vi "CIF_Iceoryx_Tag Update Test Cases.vi"() -> (0 "error out":errorcluster, 2 "status":string, 3 "pass":bool)   [LabVIEW 2021]
uses:
  ChannelCommon/typedef/Direction.ctl
  Double/CIF_Iceoryx_Chn_Double.lvclass
  D:/dev/Packages/CIF_Channels_Core/src/Iceorxy_Channels/CIF_Iceoryx_BB/CIF_Iceoryx_BB.lvclass
  D:/dev/Packages/CIF_Channels_Core/src/CIFChannels/CIFChannels.lvclass
  ChannelCommon/typedef/New FIFO Instance Response.ctl
  CIFChannels/CIFChannels.lvclass/CIFChannels.ctl
  U64/CIF_Iceoryx_Chn_U64.lvclass
  I64/CIF_Iceoryx_Chn_I64.lvclass
  CIF_Iceoryx_BB/CIF_Iceoryx_BB.lvclass/CIF_Iceoryx_BB.ctl
  8a10abfc-3488-46de-9eab-28ae7432ccba.vi
  <vilib>/CIF Foundation/CIF Iceoryx/SubVIs/Get Path.vi
  <vilib>/CIF Foundation/CIF Iceoryx/SubVIs/Convert Error.vi
  <vilib>/CIF Foundation/CIF Iceoryx/Refnum/BB Reader from Refnum.vi
  <vilib>/CIF Foundation/CIF Iceoryx/SubVIs/Convert Error Core.vi
  ChannelCommon/ChannelCommon.lvlib
  CIFChannels/CIFChannels.lvclass
  <vilib>/CIF Foundation/CIF Iceoryx/Iceoryx.lvlib
  CIF_Iceoryx_BB/CIF_Iceoryx_BB.lvclass
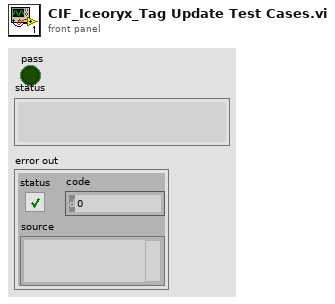
[diagram p1: front panel]
types:
  T1 = typedef "ChannelCommon.lvlib/Direction.ctl" = enum8{"Publisher", "Subscriber"}
  T2 = typedef "ChannelCommon.lvlib/New FIFO Instance Response.ctl" = cluster{"Publisher":string, "Custom Data":u8[]}
  T3 = typedef "Iceoryx.lvlib/BB Refnum.ctl" = cluster{"refnum":u64, "BB":enum8{"bb"}}
  T4 = typedef "Iceoryx.lvlib/BB Reader Refnum.ctl" = cluster{"refnum":u64, "BB Reader":enum8{"bb_reader"}}
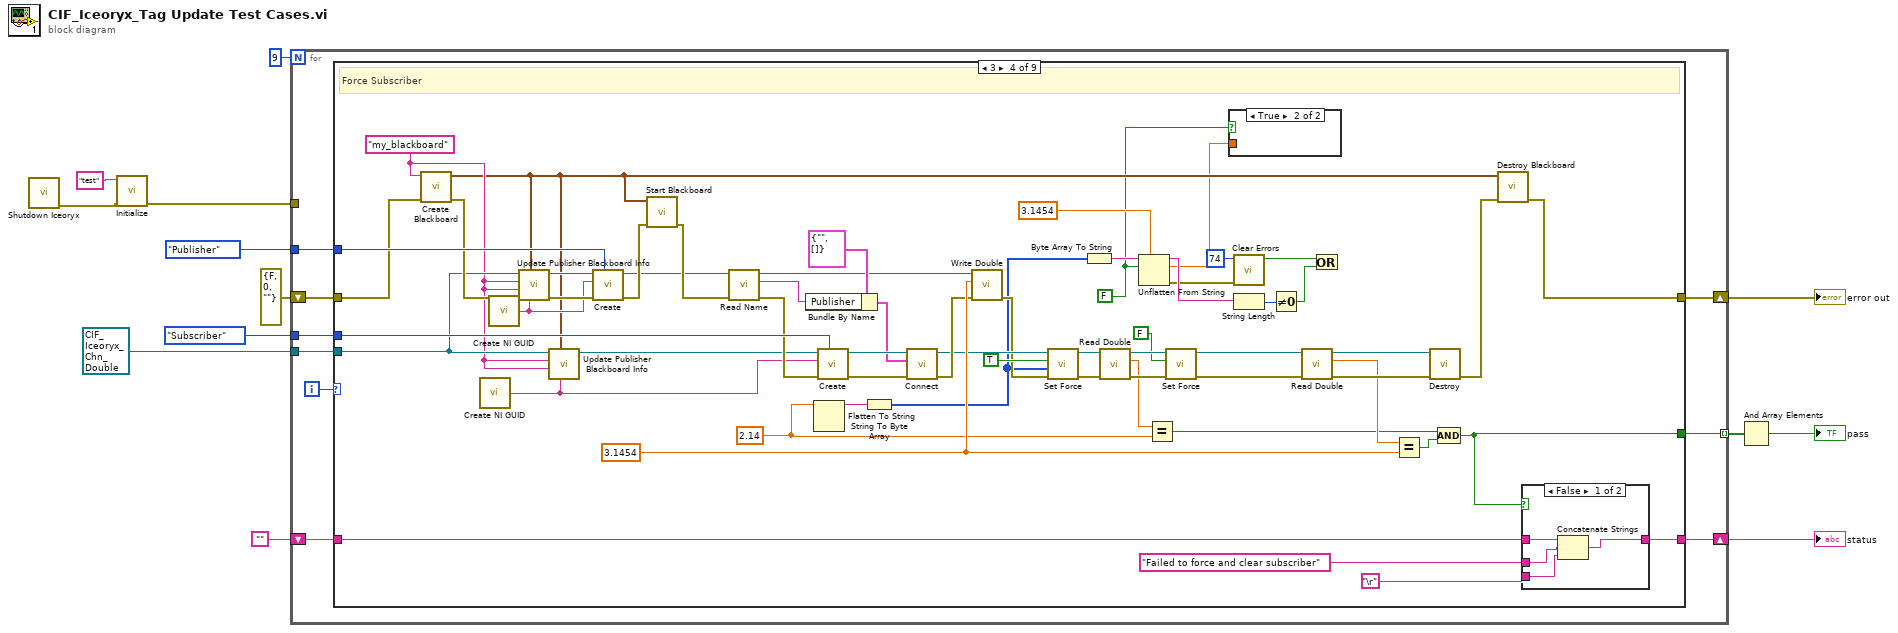
[diagram p0: block diagram]
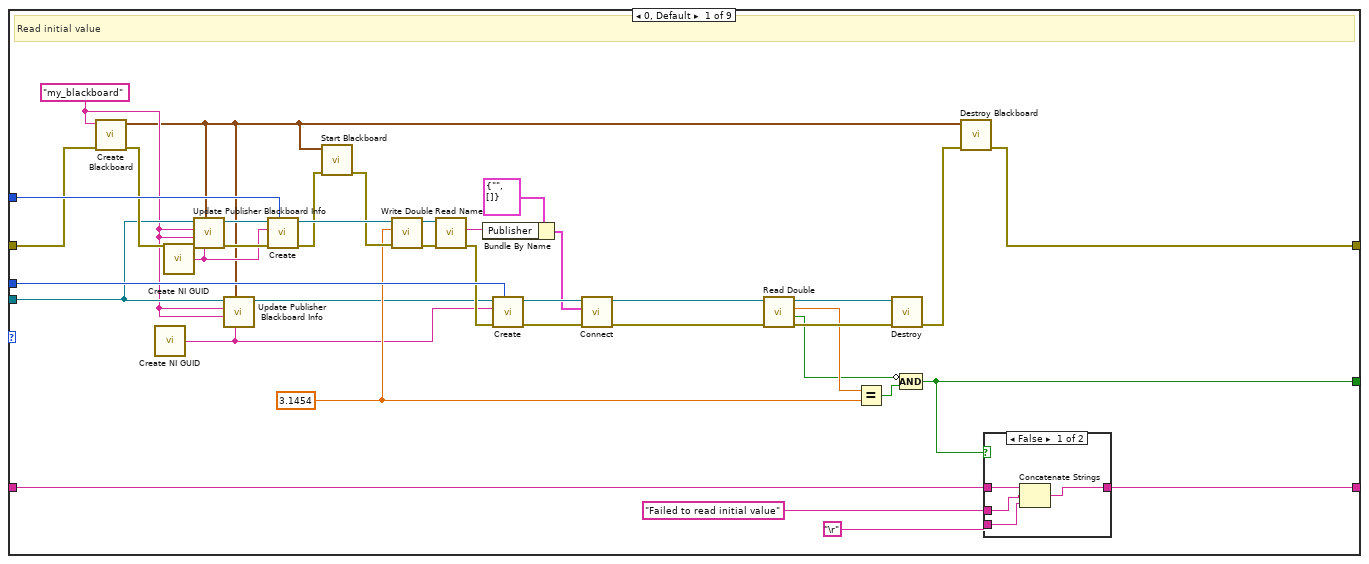
[diagram p2: hidden frame]
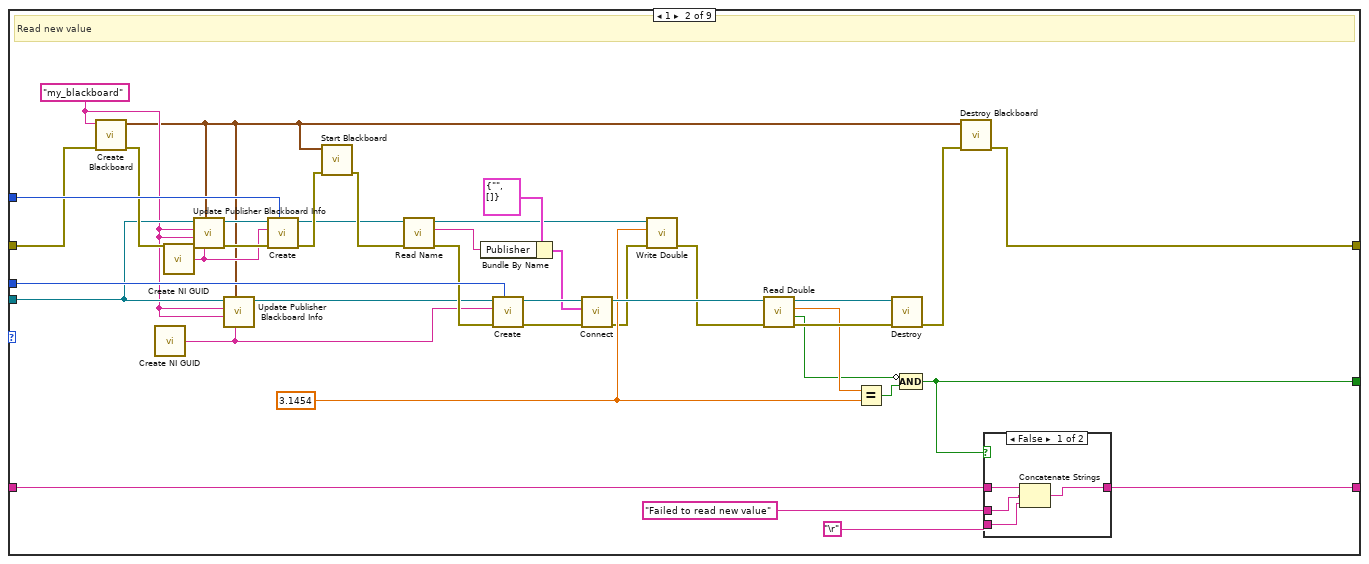
[diagram p4: hidden frame]
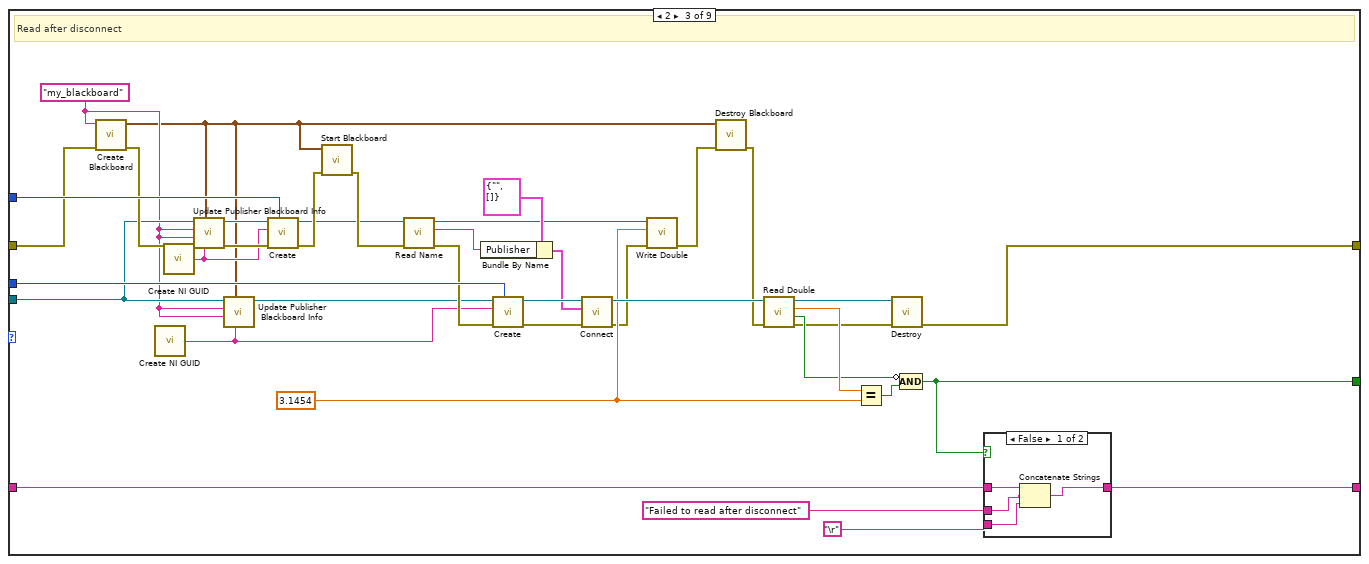
[diagram p6: hidden frame]
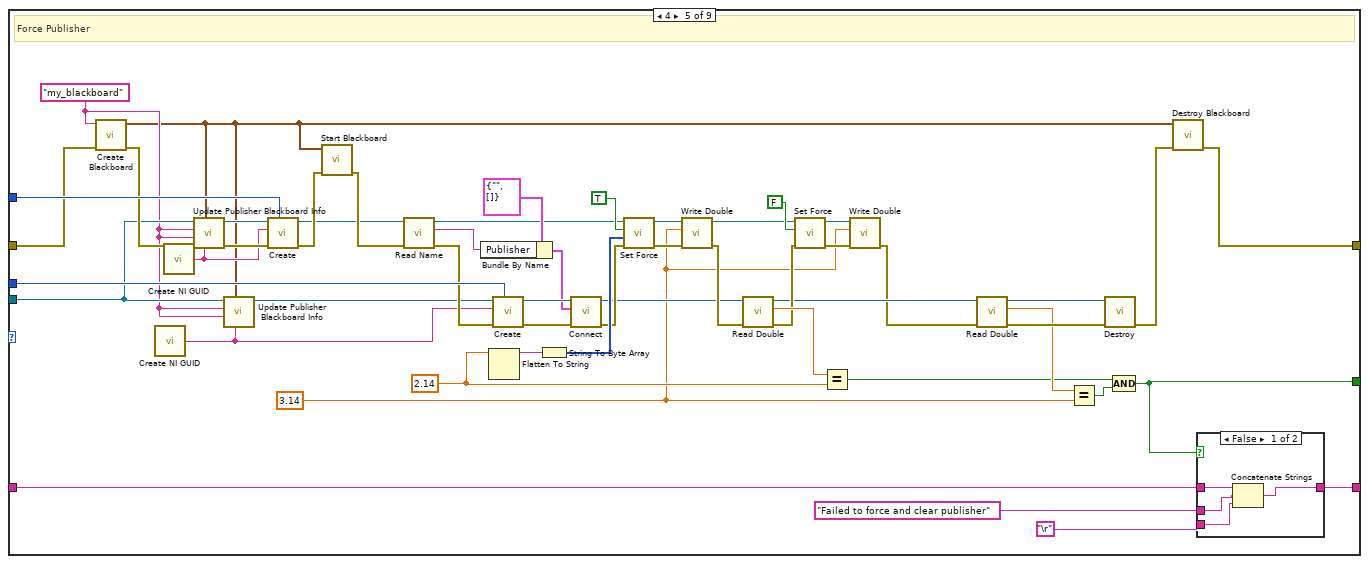
[diagram p10: hidden frame]
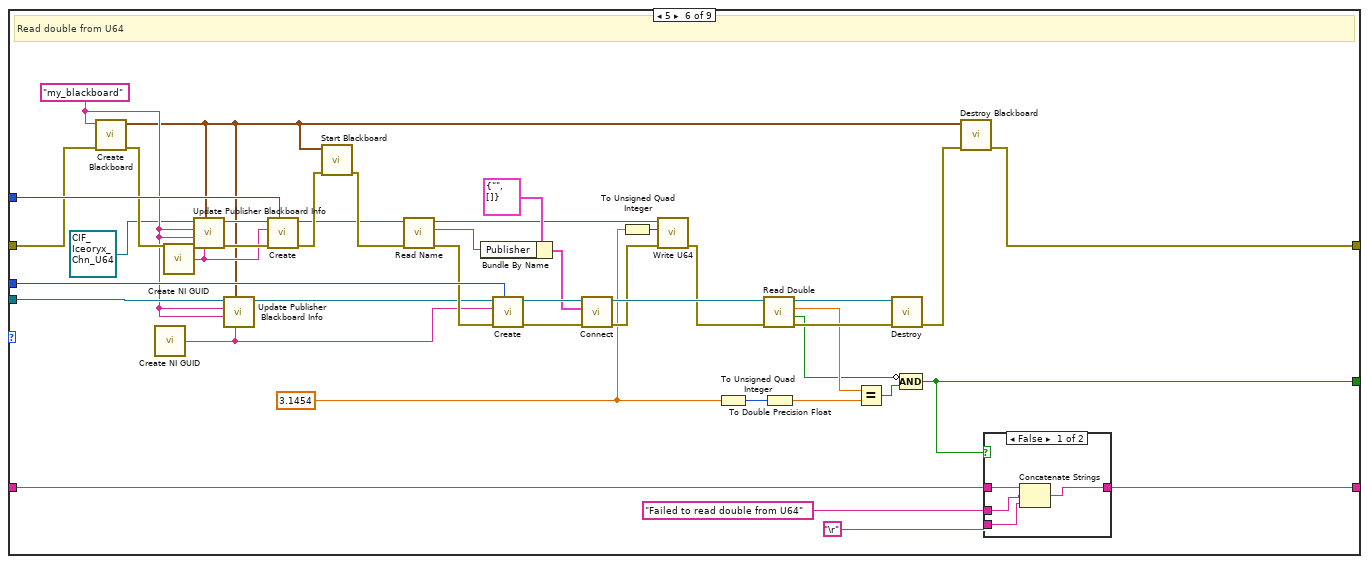
[diagram p12: hidden frame]
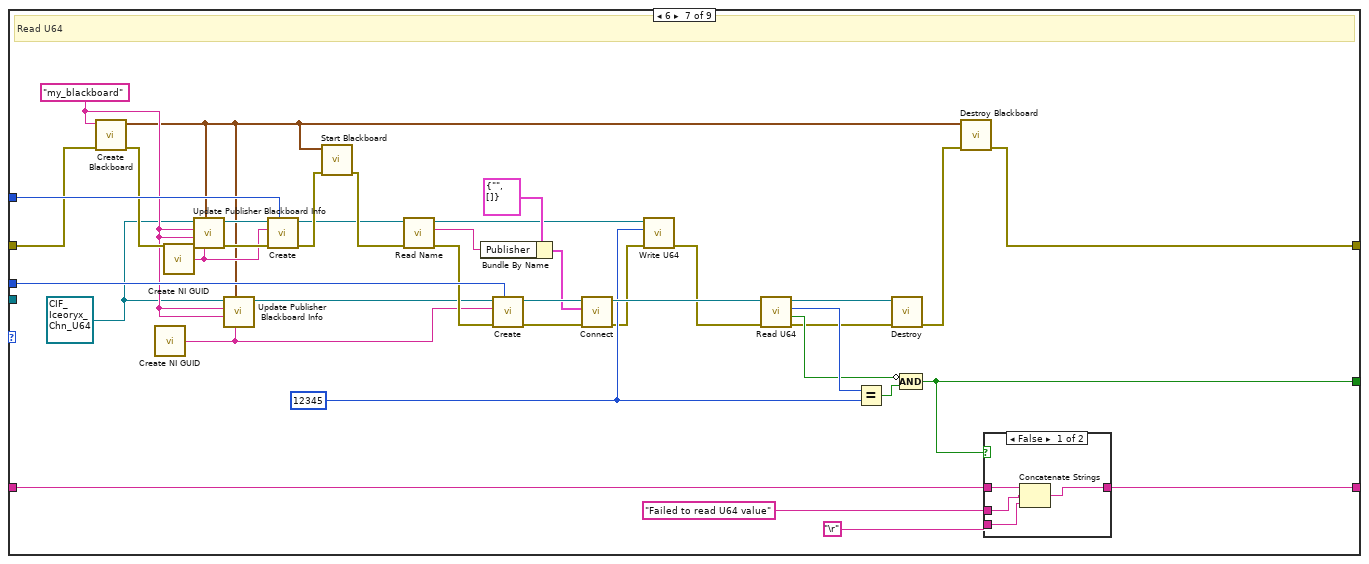
[diagram p14: hidden frame]
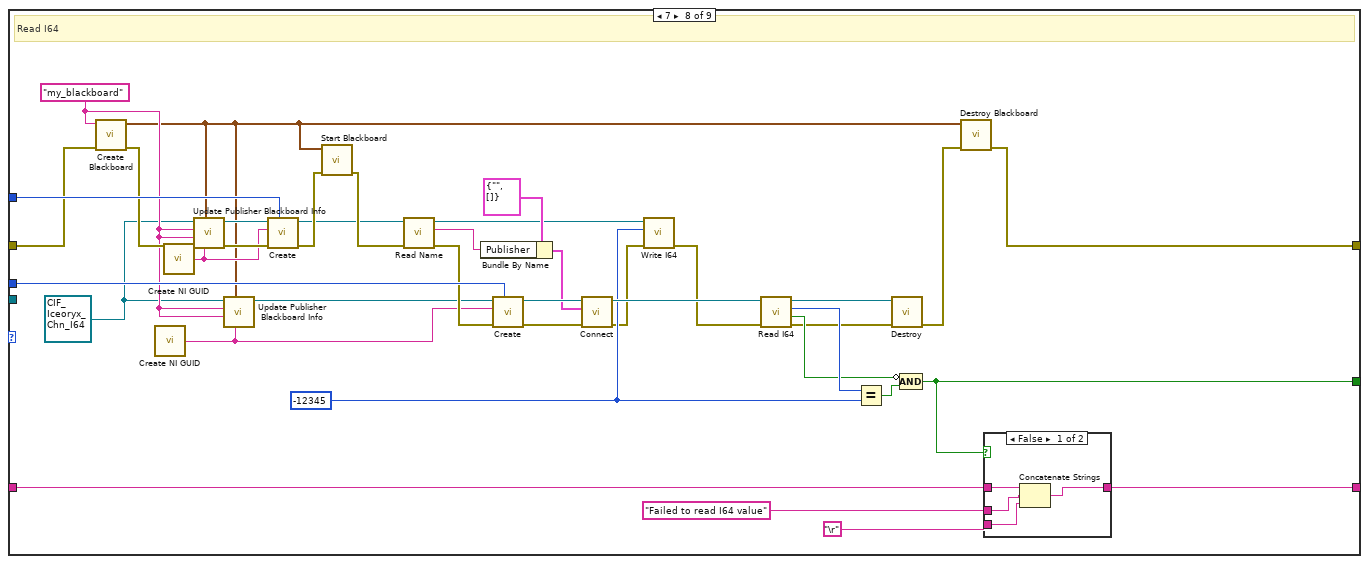
[diagram p16: hidden frame]
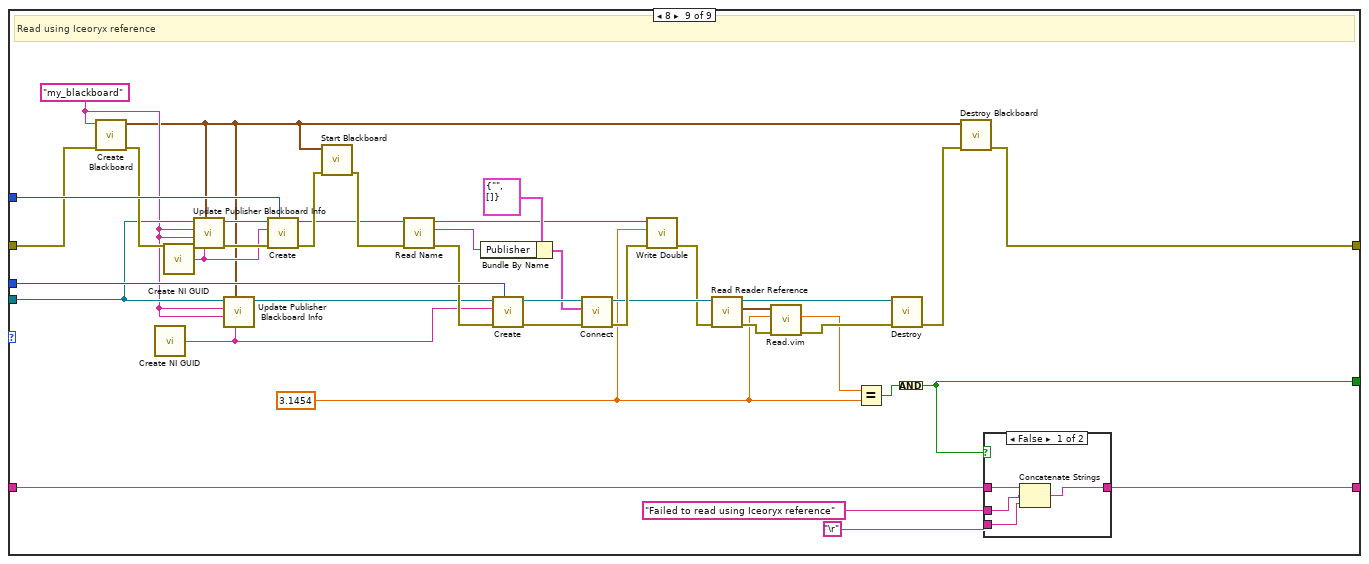
[diagram p18: hidden frame]
diagram:
  n1 = call <vilib>:"Shutdown Iceoryx.vi"() -> ("error out"=w1:errorcluster)  [unwired: 11 in]
  n2 = call <vilib>:"Initialize.vi"("error in (no error)"=w1, "Node name"="test") -> ("error out"=w2:errorcluster)  [unwired: 9 in]
  n3 = for {
    N: 9 -> [_]
    tunnel: [w22] -> w13 mode=indexing
    shift-right: [w20] -> w8
    shift-left: errorcluster {"status"=FALSE, "code"=0, "source"=""} ("error out") -> [w21]
    shift-right: [w17] -> w9
    shift-left: "" -> [w18]
    tunnel: refnum<class "CIF_Iceoryx_Chn_Double.lvclass"> refnum ("CIF_CIPC_Chn_Double.lvclass") -> [w16]
    tunnel: Direction."Publisher" ("Direction") -> [w15]
    tunnel: Direction."Subscriber" ("Direction") -> [w14]
    tunnel: w2 -> [_]
    i -> [w19]
    n4 = case shown="3" w19 {
      tunnel: [w49 w92 w136 w202 w259 w304 w351 w394 w438] -> w22
      tunnel: w21 -> [w42 w86 w130 w197 w254 w298 w346 w389 w433]
      tunnel: [w34 w79 w109 w190 w248 w292 w340 w383 w427] -> w20
      tunnel: w18 -> [w60 w103 w146 w211 w268 w315 w358 w401 w445]
      tunnel: [w59 w102 w145 w210 w267 w314 w357 w400 w444] -> w17
      tunnel: w16 -> [w27 w75 w121 w186 w244 w288 _ _ w423]
      tunnel: w15 -> [w47 w90 w134 w201 w258 w302 w350 w393 w437]
      tunnel: w14 -> [w46 w89 w133 w200 w257 w301 w349 w392 w436]
      frame 0, Default {
        w25 = "my_blackboard" ("Blackboard name")
        w39 = 3.1454
        # "Read initial value"
        n5 = call <vilib>:"Create Blackboard.vi"("error in (no error)"=w42, "Blackboard name"=w25) -> ("error out"=w38:errorcluster, "Blackboard Reference"=w23:T3)  [unwired: 8 in]
        n6 = call <vilib>:"Create NI GUID.vi"() -> ("NI GUID"=w24:string)
        n7 = call <vilib>:"Create NI GUID.vi"() -> ("NI GUID"=w32:string)
        n8 = call "Update Publisher Blackboard Info.vi"("Topic"=w32, "Blackboard Reference"=w23, "error in (no error)"=w38, "Blackboard name"=w25, "Plugin name"=w25, "CIF_Iceoryx_BB in"=w27) -> ("error out"=w37:errorcluster, "CIF_Iceoryx_BB out"=w36:refnum<class "CIF_Iceoryx_Chn_Double.lvclass">)  [unwired: 3 in, 1 out]
        n9 = call "Update Publisher Blackboard Info.vi"("Topic"=w24, "Blackboard Reference"=w23, "Blackboard name"=w25, "Plugin name"=w25, "CIF_Iceoryx_BB in"=w27) -> ("CIF_Iceoryx_BB out"=w26:refnum<class "CIF_Iceoryx_Chn_Double.lvclass">)  [unwired: 4 in, 2 out]
        n10 = call-dynamic "Create.vi"("Direction"=w47, "error in (no error)"=w37, "Name"=w32, "CIF_Iceoryx_BB in"=w36) -> ("error out"=w41:errorcluster, "CIF_Iceoryx_BB out"=w45:refnum<class "CIF_Iceoryx_Chn_Double.lvclass">)  [unwired: 6 in]
        n11 = call <vilib>:"Start Blackboard.vi"("error in (no error)"=w41, "Blackboard Reference"=w23) -> ("error out"=w40:errorcluster)  [unwired: 9 in]
        n12 = call-dynamic "Write Double.vi"("error in (no error)"=w40, "Data"=w39, "CIFTag in"=w45) -> ("error out"=w31:errorcluster, "CIFTag out"=w30:refnum<class "CIF_Iceoryx_Chn_Double.lvclass">)  [unwired: 6 in, 1 out]
        n13 = call "Read Name.vi"("error in (no error)"=w31, "CIFChannels in"=w30) -> ("error out"=w28:errorcluster, "Name"=w29:string)  [unwired: 7 in, 1 out]
        n14 = Bundle By Name(cluster=T2 {"Publisher"="", "Custom Data"=[]} ("Connection"), "Publisher"=w29) -> (w43:T2)
        n15 = call-dynamic "Create.vi"("Direction"=w46, "error in (no error)"=w28, "Name"=w24, "CIF_Iceoryx_BB in"=w26) -> ("error out"=w55:errorcluster, "CIF_Iceoryx_BB out"=w56:refnum<class "CIF_Iceoryx_Chn_Double.lvclass">)  [unwired: 6 in]
        n16 = call-dynamic "Connect.vi"("error in (no error)"=w55, "Connection"=w43, "CIF_Iceoryx_BB"=w56) -> ("error out"=w33:errorcluster, "CIF_Iceoryx_BB"=w54:refnum<class "CIF_Iceoryx_Chn_Double.lvclass">)  [unwired: 7 in]
        n17 = call-dynamic "Read Double.vi"("error in (no error)"=w33, "CIFTag in"=w54) -> ("error out"=w52:errorcluster, "timed out?"=w48:bool, "Data"=w51:dbl, "CIFTag out"=w53:refnum<class "CIF_Iceoryx_Chn_Double.lvclass">)  [unwired: 6 in]
        n18 = Equal?(x=w51, y=w39) -> (x = y?=w50:bool)
        n19 = call-dynamic "Destroy.vi"("error in (no error)"=w52, "CIF_Iceoryx_BB in"=w53) -> ("error out"=w35:errorcluster)  [unwired: 8 in, 1 out]
        n20 = Compound Arithmetic op=AND(invert w48, w50) -> (w49:bool)
        n21 = call <vilib>:"Destroy Blackboard.vi"("error in (no error)"=w35, "Blackboard Reference"=w23) -> ("error out"=w34:errorcluster)  [unwired: 8 in, 1 out]
        n22 = case shown="False" w49 {
          tunnel: w60 -> [w64 w65]
          tunnel: [w61 w65] -> w59
          tunnel: "Failed to read initial value" -> [w63 _]
          tunnel: "\r" -> [w62 _]
          frame False {
            n23 = Concatenate Strings(w64, w63, w62) -> (w61:string)
          }
          frame True {
          }
        }
      }
      frame 1 {
        w73 = "my_blackboard" ("Blackboard name")
        w84 = 3.1454
        # "Read new value"
        n24 = call <vilib>:"Create Blackboard.vi"("error in (no error)"=w86, "Blackboard name"=w73) -> ("error out"=w83:errorcluster, "Blackboard Reference"=w71:T3)  [unwired: 8 in]
        n25 = call <vilib>:"Create NI GUID.vi"() -> ("NI GUID"=w72:string)
        n26 = call <vilib>:"Create NI GUID.vi"() -> ("NI GUID"=w78:string)
        n27 = call "Update Publisher Blackboard Info.vi"("Topic"=w78, "Blackboard Reference"=w71, "error in (no error)"=w83, "Blackboard name"=w73, "Plugin name"=w73, "CIF_Iceoryx_BB in"=w75) -> ("error out"=w82:errorcluster, "CIF_Iceoryx_BB out"=w81:refnum<class "CIF_Iceoryx_Chn_Double.lvclass">)  [unwired: 3 in, 1 out]
        n28 = call "Update Publisher Blackboard Info.vi"("Topic"=w72, "Blackboard Reference"=w71, "Blackboard name"=w73, "Plugin name"=w73, "CIF_Iceoryx_BB in"=w75) -> ("CIF_Iceoryx_BB out"=w74:refnum<class "CIF_Iceoryx_Chn_Double.lvclass">)  [unwired: 4 in, 2 out]
        n29 = call-dynamic "Create.vi"("Direction"=w90, "error in (no error)"=w82, "Name"=w78, "CIF_Iceoryx_BB in"=w81) -> ("error out"=w85:errorcluster, "CIF_Iceoryx_BB out"=w68:refnum<class "CIF_Iceoryx_Chn_Double.lvclass">)  [unwired: 6 in]
        n30 = call <vilib>:"Start Blackboard.vi"("error in (no error)"=w85, "Blackboard Reference"=w71) -> ("error out"=w69:errorcluster)  [unwired: 9 in]
        n31 = call "Read Name.vi"("error in (no error)"=w69, "CIFChannels in"=w68) -> ("error out"=w76:errorcluster, "Name"=w77:string, "CIFChannels out"=w70:refnum<class "CIF_Iceoryx_Chn_Double.lvclass">)  [unwired: 7 in]
        n32 = Bundle By Name(cluster=T2 {"Publisher"="", "Custom Data"=[]} ("Connection"), "Publisher"=w77) -> (w87:T2)
        n33 = call-dynamic "Create.vi"("Direction"=w89, "error in (no error)"=w76, "Name"=w72, "CIF_Iceoryx_BB in"=w74) -> ("error out"=w98:errorcluster, "CIF_Iceoryx_BB out"=w99:refnum<class "CIF_Iceoryx_Chn_Double.lvclass">)  [unwired: 6 in]
        n34 = call-dynamic "Connect.vi"("error in (no error)"=w98, "Connection"=w87, "CIF_Iceoryx_BB"=w99) -> ("error out"=w67:errorcluster, "CIF_Iceoryx_BB"=w97:refnum<class "CIF_Iceoryx_Chn_Double.lvclass">)  [unwired: 7 in]
        n35 = call-dynamic "Write Double.vi"("error in (no error)"=w67, "Data"=w84, "CIFTag in"=w70) -> ("error out"=w66:errorcluster)  [unwired: 6 in, 2 out]
        n36 = call-dynamic "Read Double.vi"("error in (no error)"=w66, "CIFTag in"=w97) -> ("error out"=w95:errorcluster, "timed out?"=w91:bool, "Data"=w94:dbl, "CIFTag out"=w96:refnum<class "CIF_Iceoryx_Chn_Double.lvclass">)  [unwired: 6 in]
        n37 = Equal?(x=w94, y=w84) -> (x = y?=w93:bool)
        n38 = call-dynamic "Destroy.vi"("error in (no error)"=w95, "CIF_Iceoryx_BB in"=w96) -> ("error out"=w80:errorcluster)  [unwired: 8 in, 1 out]
        n39 = Compound Arithmetic op=AND(invert w91, w93) -> (w92:bool)
        n40 = call <vilib>:"Destroy Blackboard.vi"("error in (no error)"=w80, "Blackboard Reference"=w71) -> ("error out"=w79:errorcluster)  [unwired: 8 in, 1 out]
        n41 = case shown="False" w92 {
          tunnel: w103 -> [w107 w108]
          tunnel: [w104 w108] -> w102
          tunnel: "Failed to read new value" -> [w106 _]
          tunnel: "\r" -> [w105 _]
          frame False {
            n42 = Concatenate Strings(w107, w106, w105) -> (w104:string)
          }
          frame True {
          }
        }
      }
      frame 2 {
        w119 = "my_blackboard" ("Blackboard name")
        w128 = 3.1454
        # "Read after disconnect"
        n43 = call <vilib>:"Create Blackboard.vi"("error in (no error)"=w130, "Blackboard name"=w119) -> ("error out"=w127:errorcluster, "Blackboard Reference"=w117:T3)  [unwired: 8 in]
        n44 = call <vilib>:"Create NI GUID.vi"() -> ("NI GUID"=w118:string)
        n45 = call <vilib>:"Create NI GUID.vi"() -> ("NI GUID"=w124:string)
        n46 = call "Update Publisher Blackboard Info.vi"("Topic"=w124, "Blackboard Reference"=w117, "error in (no error)"=w127, "Blackboard name"=w119, "Plugin name"=w119, "CIF_Iceoryx_BB in"=w121) -> ("error out"=w126:errorcluster, "CIF_Iceoryx_BB out"=w125:refnum<class "CIF_Iceoryx_Chn_Double.lvclass">)  [unwired: 3 in, 1 out]
        n47 = call "Update Publisher Blackboard Info.vi"("Topic"=w118, "Blackboard Reference"=w117, "Blackboard name"=w119, "Plugin name"=w119, "CIF_Iceoryx_BB in"=w121) -> ("CIF_Iceoryx_BB out"=w120:refnum<class "CIF_Iceoryx_Chn_Double.lvclass">)  [unwired: 4 in, 2 out]
        n48 = call-dynamic "Create.vi"("Direction"=w134, "error in (no error)"=w126, "Name"=w124, "CIF_Iceoryx_BB in"=w125) -> ("error out"=w129:errorcluster, "CIF_Iceoryx_BB out"=w114:refnum<class "CIF_Iceoryx_Chn_Double.lvclass">)  [unwired: 6 in]
        n49 = call <vilib>:"Start Blackboard.vi"("error in (no error)"=w129, "Blackboard Reference"=w117) -> ("error out"=w115:errorcluster)  [unwired: 9 in]
        n50 = call "Read Name.vi"("error in (no error)"=w115, "CIFChannels in"=w114) -> ("error out"=w122:errorcluster, "Name"=w123:string, "CIFChannels out"=w116:refnum<class "CIF_Iceoryx_Chn_Double.lvclass">)  [unwired: 7 in]
        n51 = Bundle By Name(cluster=T2 {"Publisher"="", "Custom Data"=[]} ("Connection"), "Publisher"=w123) -> (w131:T2)
        n52 = call-dynamic "Create.vi"("Direction"=w133, "error in (no error)"=w122, "Name"=w118, "CIF_Iceoryx_BB in"=w120) -> ("error out"=w141:errorcluster, "CIF_Iceoryx_BB out"=w142:refnum<class "CIF_Iceoryx_Chn_Double.lvclass">)  [unwired: 6 in]
        n53 = call-dynamic "Connect.vi"("error in (no error)"=w141, "Connection"=w131, "CIF_Iceoryx_BB"=w142) -> ("error out"=w113:errorcluster, "CIF_Iceoryx_BB"=w140:refnum<class "CIF_Iceoryx_Chn_Double.lvclass">)  [unwired: 7 in]
        n54 = call-dynamic "Write Double.vi"("error in (no error)"=w113, "Data"=w128, "CIFTag in"=w116) -> ("error out"=w111:errorcluster)  [unwired: 6 in, 2 out]
        n55 = call <vilib>:"Destroy Blackboard.vi"("error in (no error)"=w111, "Blackboard Reference"=w117) -> ("error out"=w110:errorcluster)  [unwired: 8 in, 1 out]
        n56 = call-dynamic "Read Double.vi"("error in (no error)"=w110, "CIFTag in"=w140) -> ("error out"=w112:errorcluster, "timed out?"=w135:bool, "Data"=w138:dbl, "CIFTag out"=w139:refnum<class "CIF_Iceoryx_Chn_Double.lvclass">)  [unwired: 6 in]
        n57 = Equal?(x=w138, y=w128) -> (x = y?=w137:bool)
        n58 = call-dynamic "Destroy.vi"("error in (no error)"=w112, "CIF_Iceoryx_BB in"=w139) -> ("error out"=w109:errorcluster)  [unwired: 8 in, 1 out]
        n59 = Compound Arithmetic op=AND(invert w135, w137) -> (w136:bool)
        n60 = case shown="False" w136 {
          tunnel: w146 -> [w150 w151]
          tunnel: [w147 w151] -> w145
          tunnel: "Failed to read after disconnect" -> [w149 _]
          tunnel: "\r" -> [w148 _]
          frame False {
            n61 = Concatenate Strings(w150, w149, w148) -> (w147:string)
          }
          frame True {
          }
        }
      }
      frame 3 {
        w152 = FALSE ("data includes array or string size? (T)")
        w165 = 2.14 ("Data")
        w184 = "my_blackboard" ("Blackboard name")
        w195 = 3.1454
        # "Force Subscriber"
        n62 = call <vilib>:"Create Blackboard.vi"("error in (no error)"=w197, "Blackboard name"=w184) -> ("error out"=w194:errorcluster, "Blackboard Reference"=w182:T3)  [unwired: 8 in]
        n63 = call <vilib>:"Create NI GUID.vi"() -> ("NI GUID"=w183:string)
        n64 = call <vilib>:"Create NI GUID.vi"() -> ("NI GUID"=w189:string)
        n65 = call "Update Publisher Blackboard Info.vi"("Topic"=w189, "Blackboard Reference"=w182, "error in (no error)"=w194, "Blackboard name"=w184, "Plugin name"=w184, "CIF_Iceoryx_BB in"=w186) -> ("error out"=w193:errorcluster, "CIF_Iceoryx_BB out"=w192:refnum<class "CIF_Iceoryx_Chn_Double.lvclass">)  [unwired: 3 in, 1 out]
        n66 = call "Update Publisher Blackboard Info.vi"("Topic"=w183, "Blackboard Reference"=w182, "Blackboard name"=w184, "Plugin name"=w184, "CIF_Iceoryx_BB in"=w186) -> ("CIF_Iceoryx_BB out"=w185:refnum<class "CIF_Iceoryx_Chn_Double.lvclass">)  [unwired: 4 in, 2 out]
        n67 = call-dynamic "Create.vi"("Direction"=w201, "error in (no error)"=w193, "Name"=w189, "CIF_Iceoryx_BB in"=w192) -> ("error out"=w196:errorcluster, "CIF_Iceoryx_BB out"=w179:refnum<class "CIF_Iceoryx_Chn_Double.lvclass">)  [unwired: 6 in]
        n68 = call <vilib>:"Start Blackboard.vi"("error in (no error)"=w196, "Blackboard Reference"=w182) -> ("error out"=w180:errorcluster)  [unwired: 9 in]
        n69 = call "Read Name.vi"("error in (no error)"=w180, "CIFChannels in"=w179) -> ("error out"=w187:errorcluster, "Name"=w188:string, "CIFChannels out"=w181:refnum<class "CIF_Iceoryx_Chn_Double.lvclass">)  [unwired: 7 in]
        n70 = Bundle By Name(cluster=T2 {"Publisher"="", "Custom Data"=[]} ("Connection"), "Publisher"=w188) -> (w198:T2)
        n71 = Flatten To String(anything=w165) -> (data string=w177:string)  [unwired: 3 in, 2 out]
        n72 = call-dynamic "Create.vi"("Direction"=w200, "error in (no error)"=w187, "Name"=w183, "CIF_Iceoryx_BB in"=w185) -> ("error out"=w206:errorcluster, "CIF_Iceoryx_BB out"=w207:refnum<class "CIF_Iceoryx_Chn_Double.lvclass">)  [unwired: 6 in]
        n73 = String To Byte Array(string=w177) -> (unsigned byte array=w156:u8[])
        n74 = call-dynamic "Connect.vi"("error in (no error)"=w206, "Connection"=w198, "CIF_Iceoryx_BB"=w207) -> ("error out"=w178:errorcluster, "CIF_Iceoryx_BB"=w175:refnum<class "CIF_Iceoryx_Chn_Double.lvclass">)  [unwired: 7 in]
        n75 = call-dynamic "Write Double.vi"("error in (no error)"=w178, "Data"=w195, "CIFTag in"=w181) -> ("error out"=w168:errorcluster)  [unwired: 6 in, 2 out]
        n76 = call "Set Force.vi"("error in (no error)"=w168, "Force Data"=w156, "Force Active"=TRUE, "CIFChannels in"=w175) -> ("error out"=w173:errorcluster, "CIFChannels out"=w174:refnum<class "CIF_Iceoryx_Chn_Double.lvclass">)  [unwired: 6 in]
        n77 = Byte Array To String(unsigned byte array=w156) -> (string=w162:string)
        n78 = call-dynamic "Read Double.vi"("error in (no error)"=w173, "CIFTag in"=w174) -> ("error out"=w171:errorcluster, "Data"=w166:dbl, "CIFTag out"=w172:refnum<class "CIF_Iceoryx_Chn_Double.lvclass">)  [unwired: 6 in, 1 out]
        n79 = Unflatten From String(type=3.1454, binary string=w162, data includes array or string size? (T)=w152) -> (rest of the binary string=w160:string, value=w153:dbl, error out=w154:errorcluster)  [unwired: 2 in]
        n80 = Equal?(x=w166, y=w165) -> (x = y?=w163:bool)
        n81 = call "Set Force.vi"("error in (no error)"=w171, "Force Active"=FALSE, "CIFChannels in"=w172) -> ("error out"=w167:errorcluster, "CIFChannels out"=w169:refnum<class "CIF_Iceoryx_Chn_Double.lvclass">)  [unwired: 7 in]
        n82 = case shown="True" w152 {
          tunnel: w153 -> [_ _]
          frame False {
          }
          frame True {
          }
        }
        n83 = call <vilib>:"Clear Errors.vi"("error in (no error)"=w154, "specific error code to clear (0: all)"=74) -> ("specific error cleared?"=w158:bool)  [unwired: 4 in, 1 out]
        n84 = String Length(string=w160) -> (length=w159:i32)
        n85 = Not Equal To 0?(x=w159) -> (x != 0?=w157:bool)
        n86 = call-dynamic "Read Double.vi"("error in (no error)"=w167, "CIFTag in"=w169) -> ("error out"=w204:errorcluster, "Data"=w203:dbl, "CIFTag out"=w205:refnum<class "CIF_Iceoryx_Chn_Double.lvclass">)  [unwired: 6 in, 1 out]
        n87 = Or(x=w158, y=w157) -> ()  [unwired: 1 out]
        n88 = Equal?(x=w203, y=w195) -> (x = y?=w164:bool)
        n89 = call-dynamic "Destroy.vi"("error in (no error)"=w204, "CIF_Iceoryx_BB in"=w205) -> ("error out"=w191:errorcluster)  [unwired: 8 in, 1 out]
        n90 = Compound Arithmetic op=AND(w163, w164) -> (w202:bool)
        n91 = call <vilib>:"Destroy Blackboard.vi"("error in (no error)"=w191, "Blackboard Reference"=w182) -> ("error out"=w190:errorcluster)  [unwired: 8 in, 1 out]
        n92 = case shown="False" w202 {
          tunnel: w211 -> [w215 w216]
          tunnel: [w212 w216] -> w210
          tunnel: "Failed to force and clear subscriber" -> [w214 _]
          tunnel: "\r" -> [w213 _]
          frame False {
            n93 = Concatenate Strings(w215, w214, w213) -> (w212:string)
          }
          frame True {
          }
        }
      }
      frame 4 {
        w232 = 2.14 ("Data")
        w242 = "my_blackboard" ("Blackboard name")
        w219 = 3.14
        # "Force Publisher"
        n94 = call <vilib>:"Create Blackboard.vi"("error in (no error)"=w254, "Blackboard name"=w242) -> ("error out"=w252:errorcluster, "Blackboard Reference"=w240:T3)  [unwired: 8 in]
        n95 = call <vilib>:"Create NI GUID.vi"() -> ("NI GUID"=w241:string)
        n96 = call <vilib>:"Create NI GUID.vi"() -> ("NI GUID"=w247:string)
        n97 = call "Update Publisher Blackboard Info.vi"("Topic"=w247, "Blackboard Reference"=w240, "error in (no error)"=w252, "Blackboard name"=w242, "Plugin name"=w242, "CIF_Iceoryx_BB in"=w244) -> ("error out"=w251:errorcluster, "CIF_Iceoryx_BB out"=w250:refnum<class "CIF_Iceoryx_Chn_Double.lvclass">)  [unwired: 3 in, 1 out]
        n98 = call "Update Publisher Blackboard Info.vi"("Topic"=w241, "Blackboard Reference"=w240, "Blackboard name"=w242, "Plugin name"=w242, "CIF_Iceoryx_BB in"=w244) -> ("CIF_Iceoryx_BB out"=w243:refnum<class "CIF_Iceoryx_Chn_Double.lvclass">)  [unwired: 4 in, 2 out]
        n99 = call-dynamic "Create.vi"("Direction"=w258, "error in (no error)"=w251, "Name"=w247, "CIF_Iceoryx_BB in"=w250) -> ("error out"=w253:errorcluster, "CIF_Iceoryx_BB out"=w238:refnum<class "CIF_Iceoryx_Chn_Double.lvclass">)  [unwired: 6 in]
        n100 = call <vilib>:"Start Blackboard.vi"("error in (no error)"=w253, "Blackboard Reference"=w240) -> ("error out"=w239:errorcluster)  [unwired: 9 in]
        n101 = call "Read Name.vi"("error in (no error)"=w239, "CIFChannels in"=w238) -> ("error out"=w245:errorcluster, "Name"=w246:string, "CIFChannels out"=w229:refnum<class "CIF_Iceoryx_Chn_Double.lvclass">)  [unwired: 7 in]
        n102 = Bundle By Name(cluster=T2 {"Publisher"="", "Custom Data"=[]} ("Connection"), "Publisher"=w246) -> (w255:T2)
        n103 = Flatten To String(anything=w232) -> (data string=w237:string)  [unwired: 3 in, 2 out]
        n104 = call-dynamic "Create.vi"("Direction"=w257, "error in (no error)"=w245, "Name"=w241, "CIF_Iceoryx_BB in"=w243) -> ("error out"=w263:errorcluster, "CIF_Iceoryx_BB out"=w264:refnum<class "CIF_Iceoryx_Chn_Double.lvclass">)  [unwired: 6 in]
        n105 = String To Byte Array(string=w237) -> (unsigned byte array=w236:u8[])
        n106 = call-dynamic "Connect.vi"("error in (no error)"=w263, "Connection"=w255, "CIF_Iceoryx_BB"=w264) -> ("error out"=w227:errorcluster, "CIF_Iceoryx_BB"=w223:refnum<class "CIF_Iceoryx_Chn_Double.lvclass">)  [unwired: 7 in]
        n107 = call "Set Force.vi"("error in (no error)"=w227, "Force Data"=w236, "Force Active"=TRUE, "CIFChannels in"=w229) -> ("error out"=w226:errorcluster, "CIFChannels out"=w228:refnum<class "CIF_Iceoryx_Chn_Double.lvclass">)  [unwired: 6 in]
        n108 = call-dynamic "Write Double.vi"("error in (no error)"=w226, "Data"=w219, "CIFTag in"=w228) -> ("error out"=w224:errorcluster, "CIFTag out"=w225:refnum<class "CIF_Iceoryx_Chn_Double.lvclass">)  [unwired: 6 in, 1 out]
        n109 = call-dynamic "Read Double.vi"("error in (no error)"=w224, "CIFTag in"=w223) -> ("error out"=w222:errorcluster, "Data"=w233:dbl, "CIFTag out"=w218:refnum<class "CIF_Iceoryx_Chn_Double.lvclass">)  [unwired: 6 in, 1 out]
        n110 = call "Set Force.vi"("error in (no error)"=w222, "Force Active"=FALSE, "CIFChannels in"=w225) -> ("error out"=w220:errorcluster, "CIFChannels out"=w221:refnum<class "CIF_Iceoryx_Chn_Double.lvclass">)  [unwired: 7 in]
        n111 = Equal?(x=w233, y=w232) -> (x = y?=w230:bool)
        n112 = call-dynamic "Write Double.vi"("error in (no error)"=w220, "Data"=w219, "CIFTag in"=w221) -> ("error out"=w217:errorcluster)  [unwired: 6 in, 2 out]
        n113 = call-dynamic "Read Double.vi"("error in (no error)"=w217, "CIFTag in"=w218) -> ("error out"=w261:errorcluster, "Data"=w260:dbl, "CIFTag out"=w262:refnum<class "CIF_Iceoryx_Chn_Double.lvclass">)  [unwired: 6 in, 1 out]
        n114 = Equal?(x=w260, y=w219) -> (x = y?=w231:bool)
        n115 = call-dynamic "Destroy.vi"("error in (no error)"=w261, "CIF_Iceoryx_BB in"=w262) -> ("error out"=w249:errorcluster)  [unwired: 8 in, 1 out]
        n116 = Compound Arithmetic op=AND(w230, w231) -> (w259:bool)
        n117 = call <vilib>:"Destroy Blackboard.vi"("error in (no error)"=w249, "Blackboard Reference"=w240) -> ("error out"=w248:errorcluster)  [unwired: 8 in, 1 out]
        n118 = case shown="False" w259 {
          tunnel: w268 -> [w272 w273]
          tunnel: [w269 w273] -> w267
          tunnel: "Failed to force and clear publisher" -> [w271 _]
          tunnel: "\r" -> [w270 _]
          frame False {
            n119 = Concatenate Strings(w272, w271, w270) -> (w269:string)
          }
          frame True {
          }
        }
      }
      frame 5 {
        w286 = "my_blackboard" ("Blackboard name")
        w277 = 3.1454
        # "Read double from U64"
        n120 = call <vilib>:"Create Blackboard.vi"("error in (no error)"=w298, "Blackboard name"=w286) -> ("error out"=w296:errorcluster, "Blackboard Reference"=w284:T3)  [unwired: 8 in]
        n121 = call <vilib>:"Create NI GUID.vi"() -> ("NI GUID"=w285:string)
        n122 = call <vilib>:"Create NI GUID.vi"() -> ("NI GUID"=w291:string)
        n123 = call "Update Publisher Blackboard Info.vi"("Topic"=w291, "Blackboard Reference"=w284, "error in (no error)"=w296, "Blackboard name"=w286, "Plugin name"=w286, "CIF_Iceoryx_BB in"=refnum<class "CIF_Iceoryx_Chn_U64.lvclass"> refnum ("CIF_Iceoryx_Chn_U64.lvclass")) -> ("error out"=w295:errorcluster, "CIF_Iceoryx_BB out"=w294:refnum<class "CIF_Iceoryx_Chn_U64.lvclass">)  [unwired: 3 in, 1 out]
        n124 = call "Update Publisher Blackboard Info.vi"("Topic"=w285, "Blackboard Reference"=w284, "Blackboard name"=w286, "Plugin name"=w286, "CIF_Iceoryx_BB in"=w288) -> ("CIF_Iceoryx_BB out"=w287:refnum<class "CIF_Iceoryx_Chn_Double.lvclass">)  [unwired: 4 in, 2 out]
        n125 = call-dynamic "Create.vi"("Direction"=w302, "error in (no error)"=w295, "Name"=w291, "CIF_Iceoryx_BB in"=w294) -> ("error out"=w297:errorcluster, "CIF_Iceoryx_BB out"=w282:refnum<class "CIF_Iceoryx_Chn_U64.lvclass">)  [unwired: 6 in]
        n126 = call <vilib>:"Start Blackboard.vi"("error in (no error)"=w297, "Blackboard Reference"=w284) -> ("error out"=w283:errorcluster)  [unwired: 9 in]
        n127 = call "Read Name.vi"("error in (no error)"=w283, "CIFChannels in"=w282) -> ("error out"=w289:errorcluster, "Name"=w290:string, "CIFChannels out"=w280:refnum<class "CIF_Iceoryx_Chn_U64.lvclass">)  [unwired: 7 in]
        n128 = Bundle By Name(cluster=T2 {"Publisher"="", "Custom Data"=[]} ("Connection"), "Publisher"=w290) -> (w299:T2)
        n129 = call-dynamic "Create.vi"("Direction"=w301, "error in (no error)"=w289, "Name"=w285, "CIF_Iceoryx_BB in"=w287) -> ("error out"=w310:errorcluster, "CIF_Iceoryx_BB out"=w311:refnum<class "CIF_Iceoryx_Chn_Double.lvclass">)  [unwired: 6 in]
        n130 = call-dynamic "Connect.vi"("error in (no error)"=w310, "Connection"=w299, "CIF_Iceoryx_BB"=w311) -> ("error out"=w279:errorcluster, "CIF_Iceoryx_BB"=w309:refnum<class "CIF_Iceoryx_Chn_Double.lvclass">)  [unwired: 7 in]
        n131 = To Unsigned Quad Integer(1:w277) -> (0:w276:u64)
        n132 = call-dynamic "Write U64.vi"("error in (no error)"=w279, "Data"=w276, "CIFTag in"=w280) -> ("error out"=w278:errorcluster)  [unwired: 6 in, 2 out]
        n133 = To Unsigned Quad Integer(1:w277) -> (0:w275:u64)
        n134 = call-dynamic "Read Double.vi"("error in (no error)"=w278, "CIFTag in"=w309) -> ("error out"=w307:errorcluster, "timed out?"=w303:bool, "Data"=w306:dbl, "CIFTag out"=w308:refnum<class "CIF_Iceoryx_Chn_Double.lvclass">)  [unwired: 6 in]
        n135 = To Double Precision Float(number=w275) -> (double precision float=w274:dbl)
        n136 = Equal?(x=w306, y=w274) -> (x = y?=w305:bool)
        n137 = call-dynamic "Destroy.vi"("error in (no error)"=w307, "CIF_Iceoryx_BB in"=w308) -> ("error out"=w293:errorcluster)  [unwired: 8 in, 1 out]
        n138 = Compound Arithmetic op=AND(invert w303, w305) -> (w304:bool)
        n139 = call <vilib>:"Destroy Blackboard.vi"("error in (no error)"=w293, "Blackboard Reference"=w284) -> ("error out"=w292:errorcluster)  [unwired: 8 in, 1 out]
        n140 = case shown="False" w304 {
          tunnel: w315 -> [w319 w320]
          tunnel: [w316 w320] -> w314
          tunnel: "Failed to read double from U64" -> [w318 _]
          tunnel: "\r" -> [w317 _]
          frame False {
            n141 = Concatenate Strings(w319, w318, w317) -> (w316:string)
          }
          frame True {
          }
        }
      }
      frame 6 {
        w330 = refnum<class "CIF_Iceoryx_Chn_U64.lvclass"> refnum ("CIF_Iceoryx_Chn_U64.lvclass")
        w335 = "my_blackboard" ("Blackboard name")
        w323 = u64 12345
        # "Read U64"
        n142 = call <vilib>:"Create Blackboard.vi"("error in (no error)"=w346, "Blackboard name"=w335) -> ("error out"=w344:errorcluster, "Blackboard Reference"=w333:T3)  [unwired: 8 in]
        n143 = call <vilib>:"Create NI GUID.vi"() -> ("NI GUID"=w334:string)
        n144 = call <vilib>:"Create NI GUID.vi"() -> ("NI GUID"=w339:string)
        n145 = call "Update Publisher Blackboard Info.vi"("Topic"=w339, "Blackboard Reference"=w333, "error in (no error)"=w344, "Blackboard name"=w335, "Plugin name"=w335, "CIF_Iceoryx_BB in"=w330) -> ("error out"=w343:errorcluster, "CIF_Iceoryx_BB out"=w342:refnum<class "CIF_Iceoryx_Chn_U64.lvclass">)  [unwired: 3 in, 1 out]
        n146 = call "Update Publisher Blackboard Info.vi"("Topic"=w334, "Blackboard Reference"=w333, "Blackboard name"=w335, "Plugin name"=w335, "CIF_Iceoryx_BB in"=w330) -> ("CIF_Iceoryx_BB out"=w336:refnum<class "CIF_Iceoryx_Chn_U64.lvclass">)  [unwired: 4 in, 2 out]
        n147 = call-dynamic "Create.vi"("Direction"=w350, "error in (no error)"=w343, "Name"=w339, "CIF_Iceoryx_BB in"=w342) -> ("error out"=w345:errorcluster, "CIF_Iceoryx_BB out"=w331:refnum<class "CIF_Iceoryx_Chn_U64.lvclass">)  [unwired: 6 in]
        n148 = call <vilib>:"Start Blackboard.vi"("error in (no error)"=w345, "Blackboard Reference"=w333) -> ("error out"=w332:errorcluster)  [unwired: 9 in]
        n149 = call "Read Name.vi"("error in (no error)"=w332, "CIFChannels in"=w331) -> ("error out"=w337:errorcluster, "Name"=w338:string, "CIFChannels out"=w324:refnum<class "CIF_Iceoryx_Chn_U64.lvclass">)  [unwired: 7 in]
        n150 = Bundle By Name(cluster=T2 {"Publisher"="", "Custom Data"=[]} ("Connection"), "Publisher"=w338) -> (w347:T2)
        n151 = call-dynamic "Create.vi"("Direction"=w349, "error in (no error)"=w337, "Name"=w334, "CIF_Iceoryx_BB in"=w336) -> ("error out"=w353:errorcluster, "CIF_Iceoryx_BB out"=w354:refnum<class "CIF_Iceoryx_Chn_U64.lvclass">)  [unwired: 6 in]
        n152 = call-dynamic "Connect.vi"("error in (no error)"=w353, "Connection"=w347, "CIF_Iceoryx_BB"=w354) -> ("error out"=w322:errorcluster, "CIF_Iceoryx_BB"=w329:refnum<class "CIF_Iceoryx_Chn_U64.lvclass">)  [unwired: 7 in]
        n153 = call-dynamic "Write U64.vi"("error in (no error)"=w322, "Data"=w323, "CIFTag in"=w324) -> ("error out"=w321:errorcluster)  [unwired: 6 in, 2 out]
        n154 = call-dynamic "Read U64.vi"("error in (no error)"=w321, "CIFTag in"=w329) -> ("error out"=w325:errorcluster, "timed out?"=w326:bool, "Data"=w327:u64, "CIFTag out"=w328:refnum<class "CIF_Iceoryx_Chn_U64.lvclass">)  [unwired: 6 in]
        n155 = Equal?(x=w327, y=w323) -> (x = y?=w352:bool)
        n156 = call-dynamic "Destroy.vi"("error in (no error)"=w325, "CIF_Iceoryx_BB in"=w328) -> ("error out"=w341:errorcluster)  [unwired: 8 in, 1 out]
        n157 = Compound Arithmetic op=AND(invert w326, w352) -> (w351:bool)
        n158 = call <vilib>:"Destroy Blackboard.vi"("error in (no error)"=w341, "Blackboard Reference"=w333) -> ("error out"=w340:errorcluster)  [unwired: 8 in, 1 out]
        n159 = case shown="False" w351 {
          tunnel: w358 -> [w362 w363]
          tunnel: [w359 w363] -> w357
          tunnel: "Failed to read U64 value" -> [w361 _]
          tunnel: "\r" -> [w360 _]
          frame False {
            n160 = Concatenate Strings(w362, w361, w360) -> (w359:string)
          }
          frame True {
          }
        }
      }
      frame 7 {
        w364 = refnum<class "CIF_Iceoryx_Chn_I64.lvclass"> refnum ("CIF_Iceoryx_Chn_I64.lvclass")
        w378 = "my_blackboard" ("Blackboard name")
        w367 = i64 -12345
        # "Read I64"
        n161 = call <vilib>:"Create Blackboard.vi"("error in (no error)"=w389, "Blackboard name"=w378) -> ("error out"=w387:errorcluster, "Blackboard Reference"=w376:T3)  [unwired: 8 in]
        n162 = call <vilib>:"Create NI GUID.vi"() -> ("NI GUID"=w377:string)
        n163 = call <vilib>:"Create NI GUID.vi"() -> ("NI GUID"=w382:string)
        n164 = call "Update Publisher Blackboard Info.vi"("Topic"=w382, "Blackboard Reference"=w376, "error in (no error)"=w387, "Blackboard name"=w378, "Plugin name"=w378, "CIF_Iceoryx_BB in"=w364) -> ("error out"=w386:errorcluster, "CIF_Iceoryx_BB out"=w385:refnum<class "CIF_Iceoryx_Chn_I64.lvclass">)  [unwired: 3 in, 1 out]
        n165 = call "Update Publisher Blackboard Info.vi"("Topic"=w377, "Blackboard Reference"=w376, "Blackboard name"=w378, "Plugin name"=w378, "CIF_Iceoryx_BB in"=w364) -> ("CIF_Iceoryx_BB out"=w379:refnum<class "CIF_Iceoryx_Chn_I64.lvclass">)  [unwired: 4 in, 2 out]
        n166 = call-dynamic "Create.vi"("Direction"=w393, "error in (no error)"=w386, "Name"=w382, "CIF_Iceoryx_BB in"=w385) -> ("error out"=w388:errorcluster, "CIF_Iceoryx_BB out"=w374:refnum<class "CIF_Iceoryx_Chn_I64.lvclass">)  [unwired: 6 in]
        n167 = call <vilib>:"Start Blackboard.vi"("error in (no error)"=w388, "Blackboard Reference"=w376) -> ("error out"=w375:errorcluster)  [unwired: 9 in]
        n168 = call "Read Name.vi"("error in (no error)"=w375, "CIFChannels in"=w374) -> ("error out"=w380:errorcluster, "Name"=w381:string, "CIFChannels out"=w368:refnum<class "CIF_Iceoryx_Chn_I64.lvclass">)  [unwired: 7 in]
        n169 = Bundle By Name(cluster=T2 {"Publisher"="", "Custom Data"=[]} ("Connection"), "Publisher"=w381) -> (w390:T2)
        n170 = call-dynamic "Create.vi"("Direction"=w392, "error in (no error)"=w380, "Name"=w377, "CIF_Iceoryx_BB in"=w379) -> ("error out"=w396:errorcluster, "CIF_Iceoryx_BB out"=w397:refnum<class "CIF_Iceoryx_Chn_I64.lvclass">)  [unwired: 6 in]
        n171 = call-dynamic "Connect.vi"("error in (no error)"=w396, "Connection"=w390, "CIF_Iceoryx_BB"=w397) -> ("error out"=w366:errorcluster, "CIF_Iceoryx_BB"=w373:refnum<class "CIF_Iceoryx_Chn_I64.lvclass">)  [unwired: 7 in]
        n172 = call-dynamic "Write I64.vi"("error in (no error)"=w366, "Data"=w367, "CIFTag in"=w368) -> ("error out"=w365:errorcluster)  [unwired: 6 in, 2 out]
        n173 = call-dynamic "Read I64.vi"("error in (no error)"=w365, "CIFTag in"=w373) -> ("error out"=w369:errorcluster, "timed out?"=w370:bool, "Data"=w371:i64, "CIFTag out"=w372:refnum<class "CIF_Iceoryx_Chn_I64.lvclass">)  [unwired: 6 in]
        n174 = Equal?(x=w371, y=w367) -> (x = y?=w395:bool)
        n175 = call-dynamic "Destroy.vi"("error in (no error)"=w369, "CIF_Iceoryx_BB in"=w372) -> ("error out"=w384:errorcluster)  [unwired: 8 in, 1 out]
        n176 = Compound Arithmetic op=AND(invert w370, w395) -> (w394:bool)
        n177 = call <vilib>:"Destroy Blackboard.vi"("error in (no error)"=w384, "Blackboard Reference"=w376) -> ("error out"=w383:errorcluster)  [unwired: 8 in, 1 out]
        n178 = case shown="False" w394 {
          tunnel: w401 -> [w405 w406]
          tunnel: [w402 w406] -> w400
          tunnel: "Failed to read I64 value" -> [w404 _]
          tunnel: "\r" -> [w403 _]
          frame False {
            n179 = Concatenate Strings(w405, w404, w403) -> (w402:string)
          }
          frame True {
          }
        }
      }
      frame 8 {
        w421 = "my_blackboard" ("Blackboard name")
        w410 = 3.1454
        # "Read using Iceoryx reference"
        n180 = call <vilib>:"Create Blackboard.vi"("error in (no error)"=w433, "Blackboard name"=w421) -> ("error out"=w431:errorcluster, "Blackboard Reference"=w419:T3)  [unwired: 8 in]
        n181 = call <vilib>:"Create NI GUID.vi"() -> ("NI GUID"=w420:string)
        n182 = call <vilib>:"Create NI GUID.vi"() -> ("NI GUID"=w426:string)
        n183 = call "Update Publisher Blackboard Info.vi"("Topic"=w426, "Blackboard Reference"=w419, "error in (no error)"=w431, "Blackboard name"=w421, "Plugin name"=w421, "CIF_Iceoryx_BB in"=w423) -> ("error out"=w430:errorcluster, "CIF_Iceoryx_BB out"=w429:refnum<class "CIF_Iceoryx_Chn_Double.lvclass">)  [unwired: 3 in, 1 out]
        n184 = call "Update Publisher Blackboard Info.vi"("Topic"=w420, "Blackboard Reference"=w419, "Blackboard name"=w421, "Plugin name"=w421, "CIF_Iceoryx_BB in"=w423) -> ("CIF_Iceoryx_BB out"=w422:refnum<class "CIF_Iceoryx_Chn_Double.lvclass">)  [unwired: 4 in, 2 out]
        n185 = call-dynamic "Create.vi"("Direction"=w437, "error in (no error)"=w430, "Name"=w426, "CIF_Iceoryx_BB in"=w429) -> ("error out"=w432:errorcluster, "CIF_Iceoryx_BB out"=w416:refnum<class "CIF_Iceoryx_Chn_Double.lvclass">)  [unwired: 6 in]
        n186 = call <vilib>:"Start Blackboard.vi"("error in (no error)"=w432, "Blackboard Reference"=w419) -> ("error out"=w417:errorcluster)  [unwired: 9 in]
        n187 = call "Read Name.vi"("error in (no error)"=w417, "CIFChannels in"=w416) -> ("error out"=w424:errorcluster, "Name"=w425:string, "CIFChannels out"=w418:refnum<class "CIF_Iceoryx_Chn_Double.lvclass">)  [unwired: 7 in]
        n188 = Bundle By Name(cluster=T2 {"Publisher"="", "Custom Data"=[]} ("Connection"), "Publisher"=w425) -> (w434:T2)
        n189 = call-dynamic "Create.vi"("Direction"=w436, "error in (no error)"=w424, "Name"=w420, "CIF_Iceoryx_BB in"=w422) -> ("error out"=w440:errorcluster, "CIF_Iceoryx_BB out"=w441:refnum<class "CIF_Iceoryx_Chn_Double.lvclass">)  [unwired: 6 in]
        n190 = call-dynamic "Connect.vi"("error in (no error)"=w440, "Connection"=w434, "CIF_Iceoryx_BB"=w441) -> ("error out"=w415:errorcluster, "CIF_Iceoryx_BB"=w414:refnum<class "CIF_Iceoryx_Chn_Double.lvclass">)  [unwired: 7 in]
        n191 = call-dynamic "Write Double.vi"("error in (no error)"=w415, "Data"=w410, "CIFTag in"=w418) -> ("error out"=w413:errorcluster)  [unwired: 6 in, 2 out]
        n192 = call "Read Reader Reference.vi"("error in (no error)"=w413, "CIF_Iceoryx_BB in"=w414) -> ("error out"=w411:errorcluster, "BB Reader Refnum"=w412:T4, "CIF_Iceoryx_BB out"=w409:refnum<class "CIF_Iceoryx_Chn_Double.lvclass">)  [unwired: 7 in]
        n193 = call "Read.vim"("error in (no error)"=w411, "Data In"=w410, "Reader Reference"=w412) -> ("error out"=w408:errorcluster, "Data Out"=w407:dbl)  [unwired: 6 in, 1 out]
        n194 = Equal?(x=w407, y=w410) -> (x = y?=w439:bool)
        n195 = call-dynamic "Destroy.vi"("error in (no error)"=w408, "CIF_Iceoryx_BB in"=w409) -> ("error out"=w428:errorcluster)  [unwired: 8 in, 1 out]
        n196 = Compound Arithmetic op=AND(w439) -> (w438:bool)
        n197 = call <vilib>:"Destroy Blackboard.vi"("error in (no error)"=w428, "Blackboard Reference"=w419) -> ("error out"=w427:errorcluster)  [unwired: 8 in, 1 out]
        n198 = case shown="False" w438 {
          tunnel: w445 -> [w449 w450]
          tunnel: [w446 w450] -> w444
          tunnel: "Failed to read using Iceoryx reference" -> [w448 _]
          tunnel: "\r" -> [w447 _]
          frame False {
            n199 = Concatenate Strings(w449, w448, w447) -> (w446:string)
          }
          frame True {
          }
        }
      }
    }
  }
  "error out" <- w8
  "status" <- w9
  n200 = And Array Elements(Boolean array=w13) -> (logical AND=→"pass":bool)
